vi "Move_empty.vi"(11 "数组in":string[](array[string])) -> (3 "数组out":string[](array[string]))   [LabVIEW 2025, in "G-Uart-Class.lvclass"]
uses:
  G-Uart-Class.lvclass
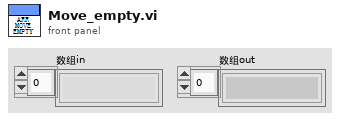
[diagram p1: front panel]
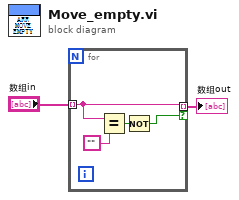
[diagram p0: block diagram]
diagram:
  n1 = for {
    tunnel: "数组in" -> [w4] mode=indexing
    tunnel: [w4] -> w1 mode=indexing if=w3
    n2 = Equal?(x=w4, y="") -> (x = y?=w5:bool)
    n3 = Not(x=w5) -> (.not. x?=w3:bool)
  }
  "数组out" <- w1
